vi "D_Check_HeadSerial.vi"(8 "error in (no error)":errorcluster, 11 "bID":u8) -> (0 "error out":errorcluster, 2 "HeadSerial":string, 3 "bID":u8, 4 "TorF":i32)   [LabVIEW 2013]
uses:
  LabVIEW2018/hpkSLMdaLV.dll
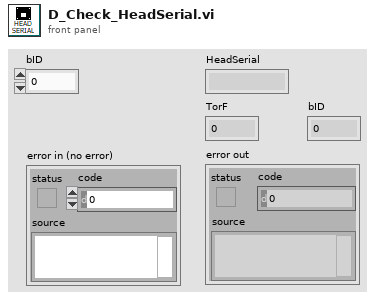
[diagram p1: front panel]
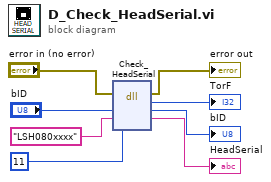
[diagram p0: block diagram]
diagram:
  n1 = dll-call lib="C:/Users/hs5921/Desktop/LabVIEW2018/hpkSLMdaLV.dll" fn="Check_HeadSerial"(error in="error in (no error)", "bID"="bID", "headSerial"="LSH080xxxx", "charSize"=11) -> (error out=→"error out":errorcluster, "返り値タイプ"=→"TorF":i32, "bID"=→"bID":u8, "headSerial"=→"HeadSerial":string)  [unwired: 3 in, 1 out]
